vi "test Parsed XML to System Definition.vi"(8 "error in":errorcluster, 11 "TestCase in":refnum<class "Scripting.lvclass">) -> (0 "error out":errorcluster, 3 "TestCase out":refnum<class "Scripting.lvclass">)   [LabVIEW 2020, in "Scripting.lvclass"]
uses:
  Scripting.lvclass
  <vilib>/addons/_JKI Toolkits/VI Tester/TestCase.llb/TestCase.lvclass
  Scripting/Ballard/Ballard ARINC 429 Scripting.lvlib
  <vilib>/NI/VeriStand Custom Device Testing Tools/VeriStandTestUtilities/VeriStandTestUtilities.lvlib
  Scripting/ARINC 429/ARINC 429 Scripting.lvlib
  Shared/VS Channels Definition for Label.ctl
  Shared/VS Channels Definition for All Labels on Hardware Channel.ctl
  <vilib>/NI/NI VeriStand Encoding and Decoding/Encoding.ctl
  <vilib>/NI/NI VeriStand Encoding and Decoding/Encoding and Decoding.lvlib
  Shared/Parameter Definition.ctl
  Shared/VS Channel Definition for Parameter.ctl
  Shared/Direction.ctl
  Shared/Transfer Type.ctl
  Shared/Transfer Speed.ctl
  C:/Program Files (x86)/National Instruments/LabVIEW 2020/vi.lib/addons/_JKI Toolkits/VI Tester/TestCase.llb/TestCase.lvclass
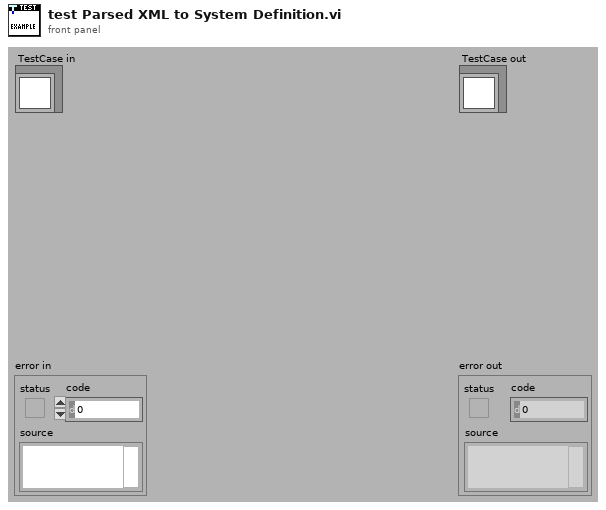
[diagram p1: front panel]
types:
  T1 = typedef "VS Channels Definition for All Labels on Hardware Channel.ctl" = cluster{"hardware channel":i32, "direction":T2, "labels":T3[], "speed":T8}
  T2 = typedef "Direction.ctl" = enum16{"Rx", "Tx"}
  T3 = typedef "VS Channels Definition for Label.ctl" = cluster{"label (Dec)":u32, "label (Display)":u32, "parameters":T4[], "SDI value":u8, "SDI enabled":bool, "transfer type":T7, "create timestamp":bool, "transmit period":u32}
  T4 = typedef "VS Channel Definition for Parameter.ctl" = cluster{"name":string, "default value":dbl, "unit":string, "Parameter":T5}
  T5 = typedef "Parameter Definition.ctl" = cluster{"start index":i32, "size":i32, "encoding":T6, "signed":bool, "scale multiplier":dbl, "scale offset":dbl}
  T6 = typedef "Encoding and Decoding.lvlib/Encoding.ctl" = enum16{"BNR", "BCD", "Discrete"}
  T7 = typedef "Transfer Type.ctl" = enum16{"Scheduled", "Acyclic", "Block", "Strobe"}
  T8 = typedef "Transfer Speed.ctl" = enum16{"LO (12.5 kb/s)", "HI (100 kb/s)"}
  T9 = typedef "Custom Device API.lvlib/Custom Device Item Ref.ctl" = u64
  T10 = typedef "Label Properties.ctl" = cluster{"label (Dec)":T11, "SDI value":u8, "SDI enabled":bool}
  T11 = typedef "Label.ctl" = u8
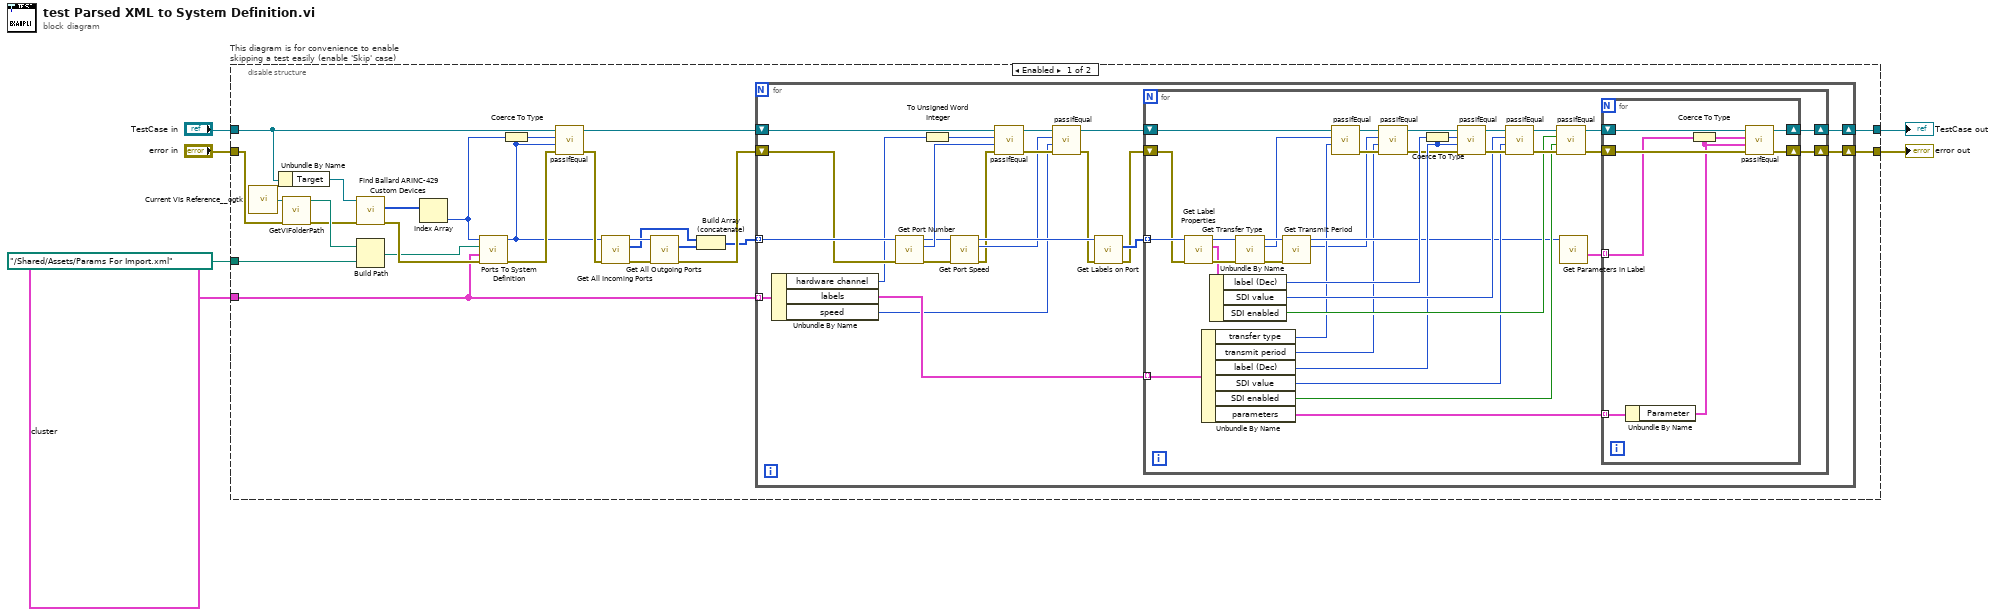
[diagram p0: block diagram]
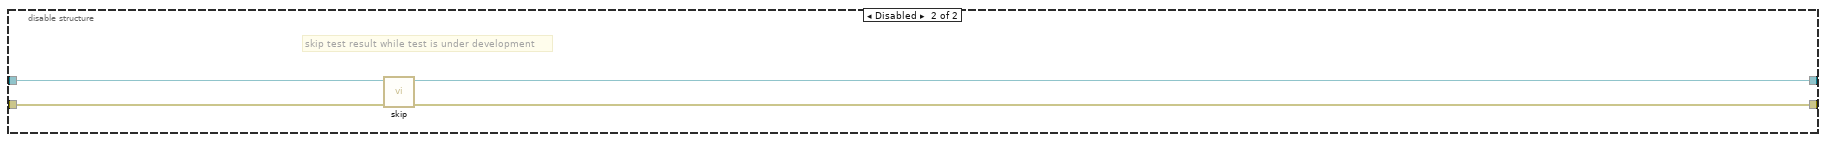
[diagram p2: hidden frame]
diagram:
  n1 = disable-structure "This diagram is for convenience to enable skipping a test easily (enable 'Skip' case)" shown="Enabled" {
    disable-tunnel: "TestCase in" -> [w24 w100]
    disable-tunnel: [w14 w98] -> w3
    disable-tunnel: [w12 w99] -> w5
    disable-tunnel: "error in" -> [w27 w97]
    disable-tunnel: T1[] [{"hardware channel"=0, "direction"=enum."Rx", "labels"=[{"label (Dec)"=134, "label (Display)"=0, "parameters"=[{"name"="Altitude_Rx", "default value"=0.0, "unit"="psi", "Parameter"={"start index"=18, "size"=10, "encoding"=enum."BNR", "signed"=TRUE, "scale multiplier"=16.0, "scale offset"=0.0}}, {"name"="SSM", "default value"=0.0, "unit"="", "Parameter"={"start index"=29, "size"=2, "encoding"=enum."BNR", "signed"=FALSE, "scale multiplier"=1.0, "scale offset"=0.0}}], "SDI value"=0, "SDI enabled"=FALSE, "transfer type"=enum."Scheduled", "create timestamp"=FALSE, "transmit period"=0}], "speed"=enum."LO (12.5 kb/s)"}, {"hardware channel"=2, "direction"=enum."Rx", "labels"=[{"label (Dec)"=135, "label (Display)"=0, "parameters"=[{"name"="Altitude_Rx", "default value"=0.0, "unit"="ft", "Parameter"={"start index"=10, "size"=19, "encoding"=enum."BCD", "signed"=TRUE, "scale multiplier"=1.0, "scale offset"=0.0}}, {"name"="SSM", "default value"=0.0, "unit"="", "Parameter"={"start index"=29, "size"=2, "encoding"=enum."BNR", "signed"=FALSE, "scale multiplier"=1.0, "scale offset"=0.0}}], "SDI value"=0, "SDI enabled"=FALSE, "transfer type"=enum."Scheduled", "create timestamp"=FALSE, "transmit period"=0}], "speed"=enum."HI (100 kb/s)"}, {"hardware channel"=4, "direction"=enum."Rx", "labels"=[{"label (Dec)"=136, "label (Display)"=0, "parameters"=[{"name"="Altitude_Rx", "default value"=0.0, "unit"="m", "Parameter"={"start index"=13, "size"=16, "encoding"=enum."BNR", "signed"=TRUE, "scale multiplier"=1.0, "scale offset"=0.0}}, {"name"="valid_Rx", "default value"=0.0, "unit"="", "Parameter"={"start index"=10, "size"=1, "encoding"=enum."Discrete", "signed"=FALSE, "scale multiplier"=1.0, "scale offset"=0.0}}, {"name"="current_Rx", "default value"=0.0, "unit"="", "Parameter"={"start index"=11, "size"=1, "encoding"=enum."Discrete", "signed"=FALSE, "scale multiplier"=1.0, "scale offset"=0.0}}, {"name"="SSM", "default value"=0.0, "unit"="", "Parameter"={"start index"=29, "size"=2, "encoding"=enum."BNR", "signed"=FALSE, "scale multiplier"=1.0, "scale offset"=0.0}}], "SDI value"=0, "SDI enabled"=FALSE, "transfer type"=enum."Scheduled", "create timestamp"=FALSE, "transmit period"=0}], "speed"=enum."HI (100 kb/s)"}, {"hardware channel"=17, "direction"=enum."Tx", "labels"=[{"label (Dec)"=134, "label (Display)"=0, "parameters"=[{"name"="Altitude_Tx", "default value"=0.0, "unit"="psi", "Parameter"={"start index"=18, "size"=10, "encoding"=enum."BNR", "signed"=TRUE, "scale multiplier"=16.0, "scale offset"=0.0}}], "SDI value"=0, "SDI enabled"=FALSE, "transfer type"=enum."Scheduled", "create timestamp"=FALSE, "transmit period"=20000}], "speed"=enum."HI (100 kb/s)"}, {"hardware channel"=19, "direction"=enum."Tx", "labels"=[{"label (Dec)"=135, "label (Display)"=0, "parameters"=[{"name"="Altitude_Tx", "default value"=0.0, "unit"="ft", "Parameter"={"start index"=10, "size"=19, "encoding"=enum."BCD", "signed"=TRUE, "scale multiplier"=1.0, "scale offset"=0.0}}], "SDI value"=0, "SDI enabled"=FALSE, "transfer type"=enum."Scheduled", "create timestamp"=FALSE, "transmit period"=0}], "speed"=enum."HI (100 kb/s)"}, {"hardware channel"=21, "direction"=enum."Tx", "labels"=[{"label (Dec)"=136, "label (Display)"=0, "parameters"=[{"name"="Altitude_Tx", "default value"=0.0, "unit"="m", "Parameter"={"start index"=13, "size"=16, "encoding"=enum."BNR", "signed"=TRUE, "scale multiplier"=1.0, "scale offset"=0.0}}, {"name"="valid_Tx", "default value"=0.0, "unit"="", "Parameter"={"start index"=10, "size"=1, "encoding"=enum."Discrete", "signed"=FALSE, "scale multiplier"=1.0, "scale offset"=0.0}}, {"name"="current_Tx", "default value"=0.0, "unit"="", "Parameter"={"start index"=11, "size"=1, "encoding"=enum."Discrete", "signed"=FALSE, "scale multiplier"=1.0, "scale offset"=0.0}}], "SDI value"=0, "SDI enabled"=FALSE, "transfer type"=enum."Acyclic", "create timestamp"=FALSE, "transmit period"=0}], "speed"=enum."LO (12.5 kb/s)"}] ("ports") -> [w8 _]
    disable-tunnel: path "../Shared/Assets/Params For Import.xml" ("Absolute or Relative Path") -> [w25 _]
    frame Enabled {
      n2 = call <userlib>:"Current VIs Reference__ogtk.vi"() -> ("Current VI's reference"=w28:refnum<vi>)  [unwired: 5 in]
      n3 = Unbundle By Name(w24) -> ("Target"=w31:refnum<k24>)
      n4 = call <vilib>:"GetVIFolderPath.vi"("error in (no error)"=w27, "VI Reference in"=w28) -> ("error out"=w26:errorcluster, "VI Folder Path out"=w29:path)  [unwired: 8 in]
      n5 = call "Find Ballard ARINC-429 Custom Devices.vi"("error in"=w26, "target in"=w31) -> ("error out"=w30:errorcluster, "Ballard ARINC 429 custom devices"=w7:u64[])  [unwired: 7 in, 1 out]
      n6 = Build Path(base path=w29, name or relative path=w25) -> (appended path=w9:path)
      n7 = Index Array(array=w7) -> (element=w22:u64)  [unwired: 1 in]
      n8 = call "Ports To System Definition.vi"("error in"=w30, "ports"=w8, "parameter configuration file path"=w9, "custom device ref"=w22) -> ("error out"=w23:errorcluster, "custom device ref out"=w10:T9)  [unwired: 6 in]
      n9 = Coerce To Type(0:w22, 1:w10) -> (2:w11:T9)
      n10 = call-dynamic "passIfEqual.vi"("error in (no error)"=w23, "y"=w10, "x"=w11, "TestCase in"=w24) -> ("error out"=w21:errorcluster, "TestCase out"=w13:refnum<class "Scripting.lvclass">)  [unwired: 6 in]
      n11 = call "Get All Incoming Ports.vi"("error in"=w21, "Ballard ARINC 429 custom device in"=w10) -> ("error out"=w19:errorcluster, "incoming ports"=w16:T9[], "Ballard ARINC 429 custom device out"=w20:T9)  [unwired: 7 in]
      n12 = call "Get All Outgoing Ports.vi"("error in"=w19, "Ballard ARINC 429 custom device in"=w20) -> ("error out"=w18:errorcluster, "outgoing ports"=w17:T9[])  [unwired: 7 in, 1 out]
      n13 = Build Array (concatenate)(w16, w17) -> (w15:T9[])
      n14 = for {
        tunnel: w15 -> [w52] mode=indexing
        tunnel: w8 -> [w53] mode=indexing
        shift-right: [w49] -> w12
        shift-left: w18 -> [w51]
        shift-right: [w43] -> w14
        shift-left: w13 -> [w46]
        n15 = Unbundle By Name(w53) -> ("hardware channel"=w45:i32, "labels"=w47:T3[], "speed"=w35:T8)
        n16 = call "Get Port Number.vi"("error in"=w51, "port ref in"=w52) -> ("error out"=w50:errorcluster, "port number"=w44:u16, "port ref out"=w41:T9)  [unwired: 6 in, 1 out]
        n17 = To Unsigned Word Integer(number=w45) -> (unsigned 16bit integer=w42:u16)
        n18 = call "Get Port Speed.vi"("error in"=w50, "port ref"=w41) -> ("error out"=w34:errorcluster, "speed"=w36:T8, "port ref out"=w40:T9)  [unwired: 7 in]
        n19 = call-dynamic "passIfEqual.vi"("error in (no error)"=w34, "y"=w44, "x"=w42, "TestCase in"=w46) -> ("error out"=w39:errorcluster, "TestCase out"=w38:refnum<class "Scripting.lvclass">)  [unwired: 6 in]
        n20 = call-dynamic "passIfEqual.vi"("error in (no error)"=w39, "y"=w35, "x"=w36, "TestCase in"=w38) -> ("error out"=w33:errorcluster, "TestCase out"=w37:refnum<class "Scripting.lvclass">)  [unwired: 6 in]
        n21 = call "Get Labels on Port.vi"("error in"=w33, "port in"=w40) -> ("error out"=w32:errorcluster, "labels"=w48:T9[])  [unwired: 6 in, 2 out]
        n22 = for {
          shift-right: [w73] -> w49
          shift-left: w32 -> [w87]
          tunnel: w48 -> [w88] mode=indexing
          tunnel: w47 -> [w85] mode=indexing
          shift-right: [w74] -> w43
          shift-left: w37 -> [w62]
          n23 = call "Get Label Properties.vi"("error in"=w87, "label ref in"=w88) -> ("error out"=w86:errorcluster, "label properties"=w84:T10, "label ref out"=w65:T9)  [unwired: 6 in, 1 out]
          n24 = Unbundle By Name(w85) -> ("transfer type"=w56:T7, "transmit period"=w54:u32, "label (Dec)"=w69:u32, "SDI value"=w70:u8, "SDI enabled"=w71:bool, "parameters"=w82:T4[])
          n25 = Unbundle By Name(w84) -> ("label (Dec)"=w68:T11, "SDI value"=w77:u8, "SDI enabled"=w72:bool)
          n26 = call "Get Transfer Type.vi"("error in"=w86, "label ref in"=w65) -> ("error out"=w66:errorcluster, "transfer type"=w57:T7, "label ref out"=w64:T9)  [unwired: 7 in]
          n27 = call "Get Transmit Period.vi"("error in"=w66, "label ref"=w64) -> ("transmit period (us)"=w55:u32, "label ref out"=w63:T9)  [unwired: 7 in, 1 out]
          n28 = call-dynamic "passIfEqual.vi"("y"=w56, "x"=w57, "TestCase in"=w62) -> ("error out"=w58:errorcluster, "TestCase out"=w61:refnum<class "Scripting.lvclass">)  [unwired: 7 in]
          n29 = call-dynamic "passIfEqual.vi"("error in (no error)"=w58, "y"=w54, "x"=w55, "TestCase in"=w61) -> ("error out"=w59:errorcluster, "TestCase out"=w60:refnum<class "Scripting.lvclass">)  [unwired: 6 in]
          n30 = Coerce To Type(0:w68, 1:w69) -> (2:w67:u32)
          n31 = call-dynamic "passIfEqual.vi"("error in (no error)"=w59, "y"=w69, "x"=w67, "TestCase in"=w60) -> ("error out"=w78:errorcluster, "TestCase out"=w79:refnum<class "Scripting.lvclass">)  [unwired: 6 in]
          n32 = call-dynamic "passIfEqual.vi"("error in (no error)"=w78, "y"=w70, "x"=w77, "TestCase in"=w79) -> ("error out"=w81:errorcluster, "TestCase out"=w80:refnum<class "Scripting.lvclass">)  [unwired: 6 in]
          n33 = call-dynamic "passIfEqual.vi"("error in (no error)"=w81, "y"=w71, "x"=w72, "TestCase in"=w80) -> ("error out"=w75:errorcluster, "TestCase out"=w76:refnum<class "Scripting.lvclass">)  [unwired: 6 in]
          n34 = call "Get Parameters in Label.vi"("label in"=w63) -> ("parameter definitions"=w83:T5[])  [unwired: 7 in, 3 out]
          n35 = for {
            tunnel: w83 -> [w93] mode=indexing
            tunnel: w82 -> [w96] mode=indexing
            shift-right: [w91] -> w74
            shift-left: w76 -> [w95]
            shift-right: [w92] -> w73
            shift-left: w75 -> [w94]
            n36 = Unbundle By Name(w96) -> ("Parameter"=w89:T5)
            n37 = Coerce To Type(0:w93, 1:w89) -> (2:w90:T5)
            n38 = call-dynamic "passIfEqual.vi"("error in (no error)"=w94, "y"=w89, "x"=w90, "TestCase in"=w95) -> ("error out"=w92:errorcluster, "TestCase out"=w91:refnum<class "Scripting.lvclass">)  [unwired: 6 in]
          }
        }
      }
    }
    frame Disabled {
      # "skip test result while test is under development"
      n39 = call <vilib>:"skip.vi"("error in (no error)"=w97, "TestCase in"=w100) -> ("error out"=w99:errorcluster, "TestCase out"=w98:refnum<class "Scripting.lvclass">)  [unwired: 8 in]
    }
  }
  "error out" <- w5
  "TestCase out" <- w3
